vi "C_Decode_RT.vi"(8 "error in (no error)":errorcluster, 10 "buffers in":T2, 11 "bytes in":u8[](array[numeric])) -> (0 "error out":errorcluster, 2 "buffers out":T2, 3 "result":T1)   [LabVIEW 2021, in "CANsub_C.lvlib"]
doc: "Real-time decode: feeds the bytes of one TCP Read into the decoder in place, in the buffers from C_RX_Buffers_Init. No allocation, no copy. The frames are in the buffer arrays at indexes 0 … n frames - 1."
uses:
  CANsub_C.lvlib
  C_Decode_Result.ctl
  codec_vis/CANsub_Codec.lvlib
  C_RX_Buffers.ctl
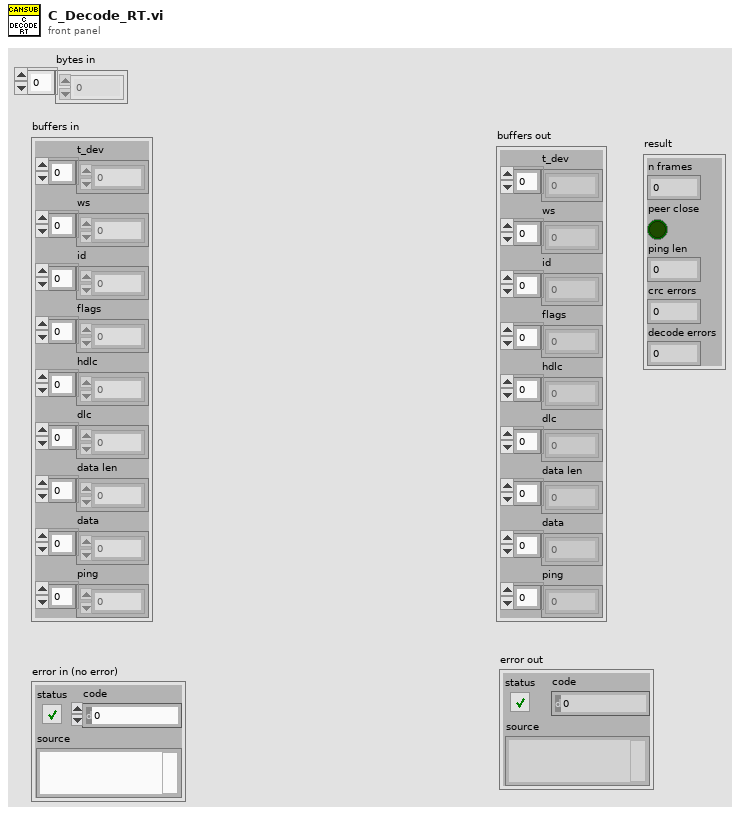
[diagram p1: front panel]
types:
  T1 = typedef "CANsub_C.lvlib/C_Decode_Result.ctl" = cluster{"n frames":i32, "peer close":bool, "ping len":i32, "crc errors":u32, "decode errors":i32}
  T2 = typedef "CANsub_C.lvlib/C_RX_Buffers.ctl" = cluster{"t_dev":dbl[], "ws":u8[], "id":u32[], "flags":u16[], "hdlc":u8[], "dlc":u8[], "data len":u8[], "data":u8[], "ping":u8[]}
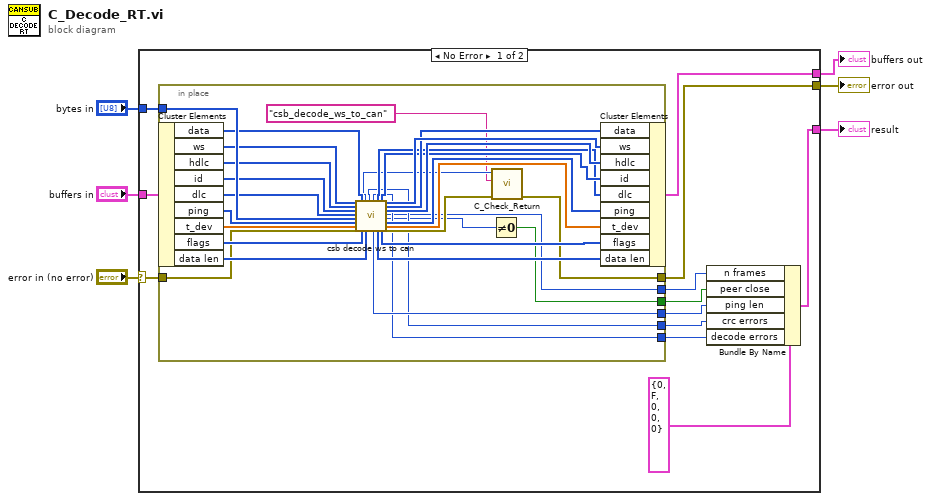
[diagram p0: block diagram]
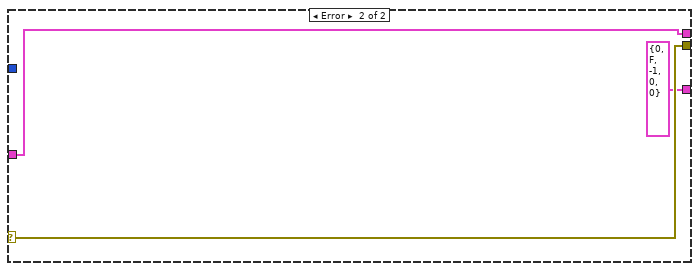
[diagram p2: hidden frame]
diagram:
  n1 = case shown="No Error" "error in (no error)" {
    selector: "error in (no error)" -> [w16 w51]
    tunnel: [w7 w51] -> w5
    tunnel: [w15 w50] -> w4
    tunnel: "buffers in" -> [w18 w50]
    tunnel: [w8 T1 {"n frames"=0, "peer close"=FALSE, "ping len"=-1, "crc errors"=0, "decode errors"=0} ("result")] -> w2
    tunnel: "bytes in" -> [w17 _]
    frame No Error {
      n2 = in-place {
        in-place-border: w17 -> [w48]
        in-place-border: w16 -> [w39]
        in-place-border: [w25] -> w13
        in-place-border: [w24] -> w12
        in-place-border: [w23] -> w11
        in-place-border: [w22] -> w10
        in-place-border: [w20] -> w9
        in-place-border: [w19] -> w7
        n3 = in-place-cluster #1(w18) -> ("data"=w37:u8[], "ws"=w47:u8[], "hdlc"=w46:u8[], "id"=w45:u32[], "dlc"=w44:u8[], "ping"=w43:u8[], "t_dev"=w42:dbl[], "flags"=w41:u16[], "data len"=w40:u8[])
        n4 = call "csb decode ws to can.vi"("ws_state"=w47, "hdlc_state"=w46, "id"=w45, "dlc"=w44, "in"=w48, "ping_payload"=w43, "t_dev"=w42, "error in (no error)"=w39, "data"=w37, "flags"=w41, "data_len"=w40) -> ("function return"=w28:i32, "crc_errors"=w24:u32, "decode_errors"=w23:i32, "ping_len"=w25:i32, "dlc out"=w29:u8[], "data_len out"=w31:u8[], "id out"=w30:u32[], "flags out"=w32:u16[], "ws_state out"=w38:u8[], "data out"=w36:u8[], "hdlc_state out"=w35:u8[], "n_frames"=w22:i32, "peer_close"=w21:i32, "ping_payload out"=w34:u8[], "t_dev out"=w33:dbl[], "error out"=w27:errorcluster)  [unwired: 1 in]
        n5 = Not Equal To 0?(x=w21) -> (x != 0?=w20:bool)
        n6 = call "C_Check_Return.vi"("error in (no error)"=w27, "function name"="csb_decode_ws_to_can", "function return"=w28) -> ("error out"=w19:errorcluster)  [unwired: 6 in, 2 out]
        n7 = in-place-cluster #1("data"=w36, "ws"=w38, "hdlc"=w35, "id"=w30, "dlc"=w29, "ping"=w34, "t_dev"=w33, "flags"=w32, "data len"=w31) -> (w15:T2)
      }
      n8 = Bundle By Name(cluster=T1 {"n frames"=0, "peer close"=FALSE, "ping len"=0, "crc errors"=0, "decode errors"=0} ("C_Decode_Result"), "n frames"=w10, "peer close"=w9, "ping len"=w13, "crc errors"=w12, "decode errors"=w11) -> (w8:T1)
    }
    frame Error {
    }
  }
  "buffers out" <- w4
  "result" <- w2
  "error out" <- w5
